vi "FPGA Acquire.vi"(0 "Logging queue in":T6, 1 "Max allowed trial length (sec)":dbl=15.0 format="%#_13g", 5 "Logging queue element IN":T3={"Imaging Protocol"=enum."Live Imaging", "Number of Trials"=0, "Frame Size"=512, "# Averaged frames"=0, "Dwell time (us)"=0.0, "Index of Z-plane"=0, "Timelapse?"=FALSE, "Logging process is active"=FALSE, "Speed logging enabled"=FALSE, "tdms file ref"=refnum, "path"=path "", "Trial Number"=0, "Expected # points acquired"=FALSE, "Manually stopped"=FALSE, "Last trial"=FALSE, "Ch0 data"=[], "Ch1 data"=[], "Ref Data"=[], "Ref Frame Time"=[], "Image Time"=[], "Continuous Time"=[], "Ref X Length"=0, "Ref Y Length"=0, "# Ref Averaged frames"=0, "Ref Dwell time (us)"=0.0, "Points acquired"={"Ch0 last trial"=0, "Ch1 last trial"=0, "All trials"=0}, "HW Timings File"=refnum} {"Ref Dwell time (us)" format="%#.6g"; "Frame Size" items=["100X100"=100, "128X128"=128, "200X200"=200, "256X256"=256, "512X512"=512, "1024x1024"=1024, "2048x2048"=2048]; "Dwell time (us)" format="%#.6g"}, 7 "FPGA Ref":T2, 9 "Target number of points":u64, 11 "error in (no error)":errorcluster, 12 "Total number of Ref points":u32, 13 "Imaging Protocol":T1) -> (4 "Logging queue out":T6, 6 "Logging queue element OUT":T3={"Imaging Protocol"=enum."Live Imaging", "Number of Trials"=0, "Frame Size"=512, "# Averaged frames"=0, "Dwell time (us)"=0.0, "Index of Z-plane"=0, "Timelapse?"=FALSE, "Logging process is active"=FALSE, "Speed logging enabled"=FALSE, "tdms file ref"=refnum, "path"=path "", "Trial Number"=0, "Expected # points acquired"=FALSE, "Manually stopped"=FALSE, "Last trial"=FALSE, "Ch0 data"=[], "Ch1 data"=[], "Ref Data"=[], "Ref Frame Time"=[], "Image Time"=[], "Continuous Time"=[], "Ref X Length"=0, "Ref Y Length"=0, "# Ref Averaged frames"=0, "Ref Dwell time (us)"=0.0, "Points acquired"={"Ch0 last trial"=0, "Ch1 last trial"=0, "All trials"=0}, "HW Timings File"=refnum} {"Ref Dwell time (us)" format="%#.6g"; "Frame Size" items=["100X100"=100, "128X128"=128, "200X200"=200, "256X256"=256, "512X512"=512, "1024x1024"=1024, "2048x2048"=2048]; "Dwell time (us)" format="%#.6g"}, 8 "Elements Remaining":u32, 10 "VI exec time":u32, 15 "error out":errorcluster)   [LabVIEW 2020]
uses:
  Typedefs/Logging queue element.ctl
  Typedefs/Imaging Protocols enum.ctl
  Typedefs/Frame Size.ctl
  Typedefs/Acquired points count.ctl
  Typedefs/Data queue ref.ctl
  RIG-SPECIFIC FILES/FPGA Refs/FPGA Ref.ctl
panel:
  out "Array":u32[](array[numeric])
  out "Ref Elements Remaining":u32
  out "# elements in queue":i32
  out "VI exec interval":u32
  out "Execution rate (Hz) 3":i32 format="Execution Rate: %.0f Hz"
  out "Execution rate (Hz)":i32 format="Execution Rate: %.0f Hz"
  out "Trial completed or \nImaging stopped":bool
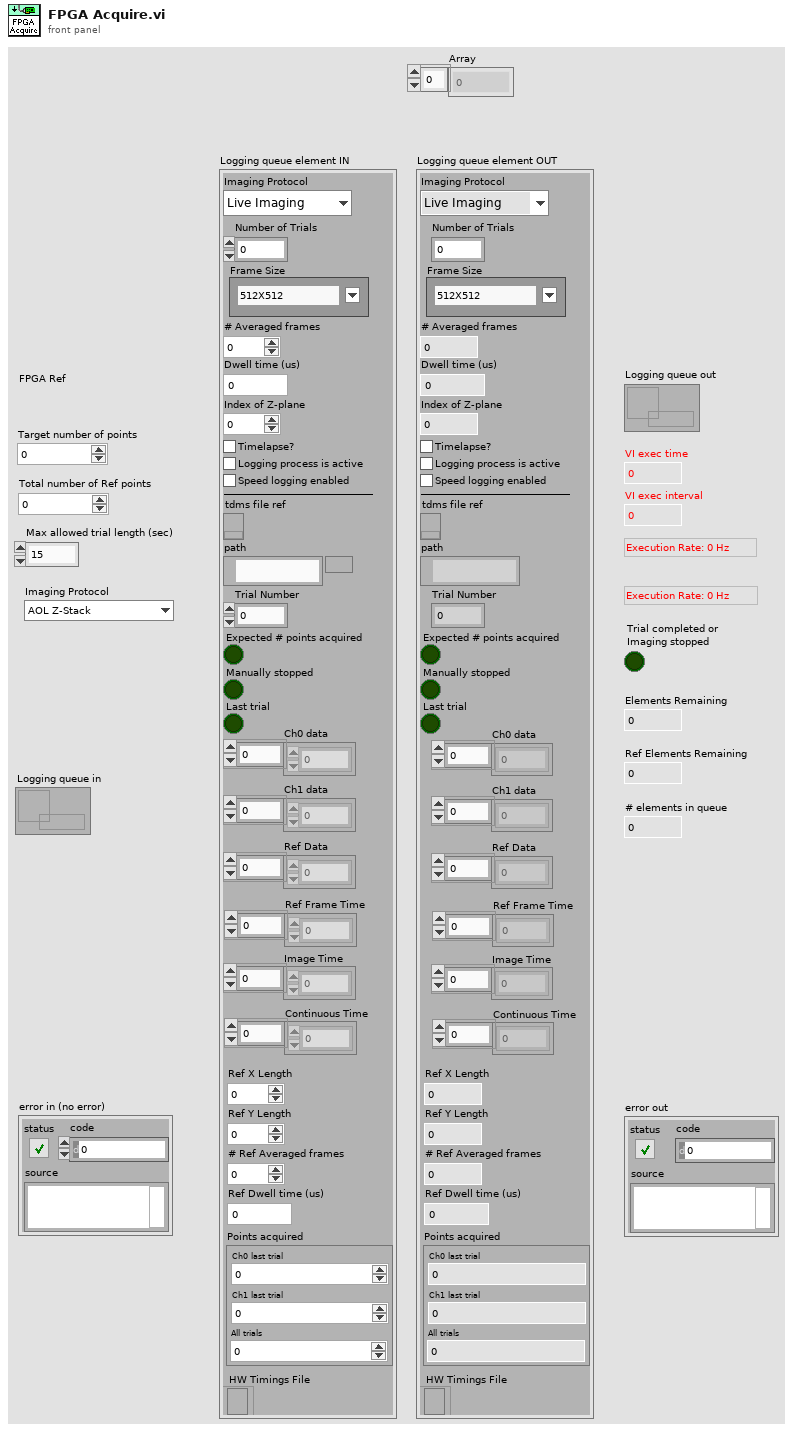
[diagram p1: front panel]
types:
  T1 = typedef "Imaging Protocols enum.ctl" = enum16{"AOL Z-Stack", "Motor Z Stack", "Functional Acquisition", "Single Plane Acquisition", "Volume Acquisition", "Live Imaging", "Live Plane Imaging", "Live Volume Imaging"}
  T2 = typedef "FPGA Ref.ctl" = refnum<k20>
  T3 = typedef "Logging queue element.ctl" = cluster{"Imaging Protocol":T1, "Number of Trials":u16, "Frame Size":T4, "# Averaged frames":u16, "Dwell time (us)":dbl, "Index of Z-plane":i32, "Timelapse?":bool, "Logging process is active":bool, "Speed logging enabled":bool, "tdms file ref":refnum<k34>, "path":path, "Trial Number":i32, "Expected # points acquired":bool, "Manually stopped":bool, "Last trial":bool, "Ch0 data":u32[], "Ch1 data":u32[], "Ref Data":u32[], "Ref Frame Time":u64[], "Image Time":u64[], "Continuous Time":u64[], "Ref X Length":u16, "Ref Y Length":u16, "# Ref Averaged frames":u16, "Ref Dwell time (us)":dbl, "Points acquired":T5, "HW Timings File":refnum<file>}
  T4 = typedef "Frame Size.ctl" = u16
  T5 = typedef "Acquired points count.ctl" = cluster{"Ch0 last trial":u64, "Ch1 last trial":u64, "All trials":u64}
  T6 = typedef "Data queue ref.ctl" = refnum<queue>
  T7 = typedef "FIFO elements available.ctl" = cluster{"Elements Available Ch0":u32, "Elements Available Ch1":u32, "Ref Elements Available":u32, "Ref Time Elements":u32, "Image Time Elements":u32, "Inter trial elements":u32, "Target number of points":u64}
  T8 = typedef "Data arrays cluster.ctl" = cluster{"Ch0 data":u32[], "Ch1 data":u32[], "Ref data":u32[], "Ref time data":u64[], "Image time data":u64[], "Continuous time data":u64[]}
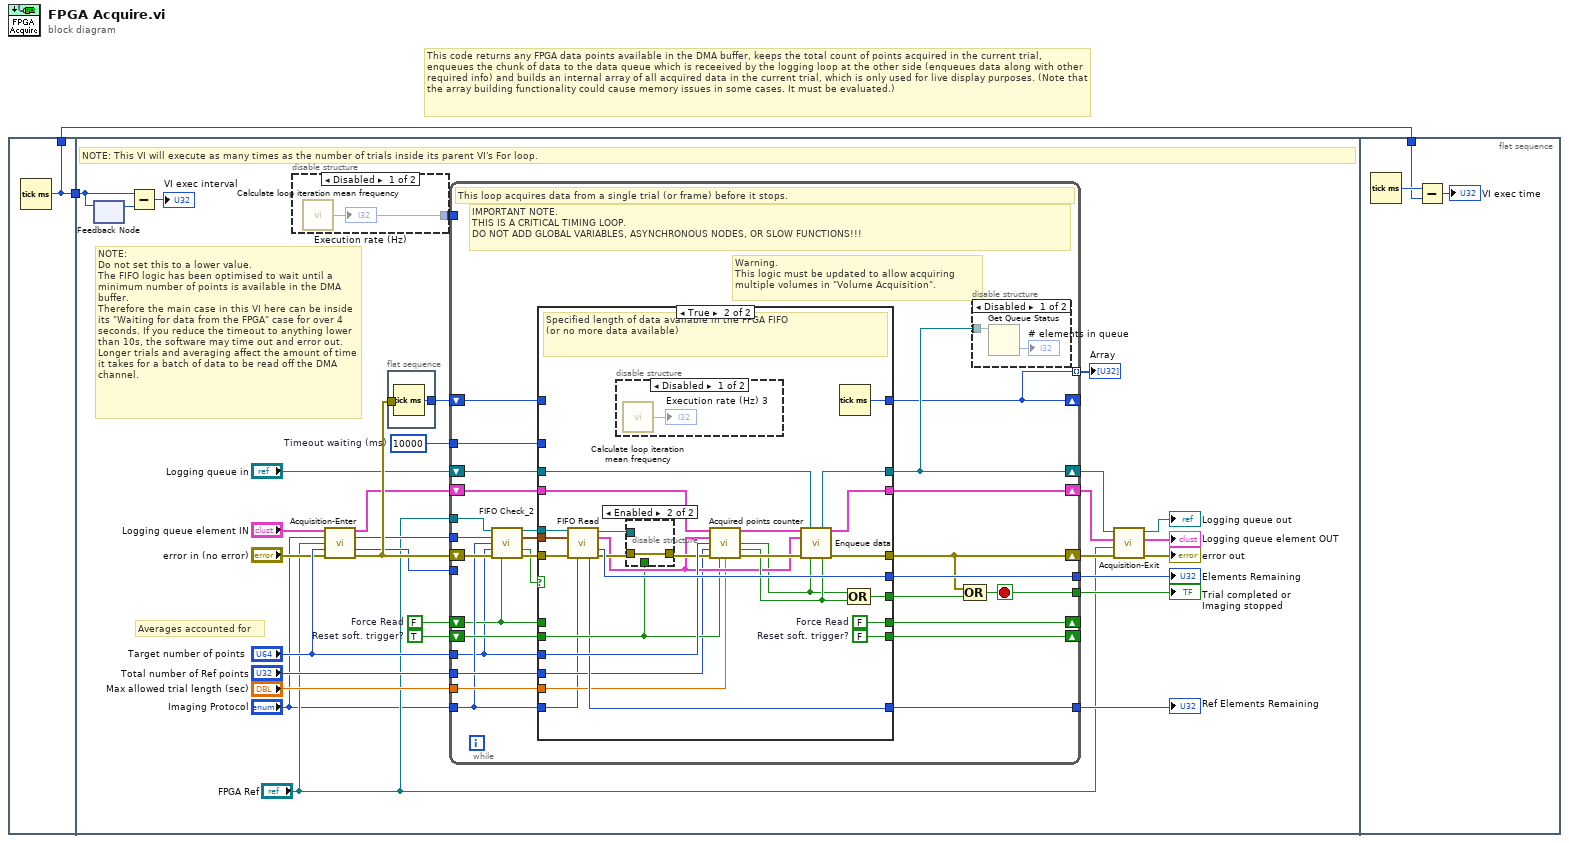
[diagram p0: block diagram]
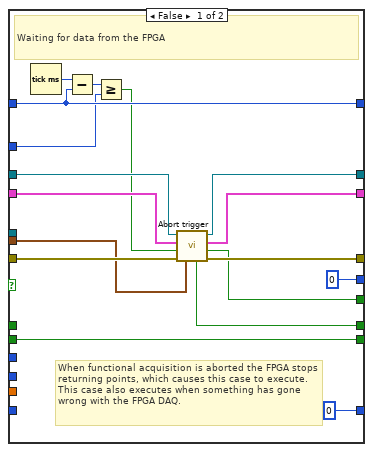
[diagram p4: hidden frame]
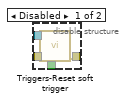
[diagram p6: hidden frame]
diagram:
  # "This code returns any FPGA data points available in the DMA buffer, keeps the total count of points acquired in the current trial, enqueues the chunk of data to the data queue which is receeived by the logging loop at the other side (enqueues data along with other required info) and builds an internal array of all acquired data in the current trial, which is only used for live display purposes. (Note that the array building functionality could cause memory issues in some cases. It must be evaluated.)"
  n1 = flat-sequence {
    tunnel: [w3] -> w1
    tunnel: [w3] -> w2
    tunnel: w2 -> [w23]
    tunnel: w1 -> [w115]
    frame #0 {
      n2 = Tick Count (ms)() -> (millisecond timer value=w3:u32)
    }
    frame #1 {
      w4 = FALSE  # Force Read
      w22 = TRUE  # Reset soft. trigger?
      w27 = u32 10000  # Timeout waiting (ms)
      # "NOTE:\nDo not set this to a lower value.\nThe FIFO logic has been optimised to wait until a minimum number of points is available in the DMA buffer.\nTherefore the main case in this VI here can be inside its \"Waiting for data from the FPGA\" case for over 4 seconds. If you reduce the timeout to anything lower than 10s, the software may time out and error out.\nLonger trials and averaging affect the amount of time it takes for a batch of data to be read off the DMA channel."
      # "Averages accounted for"
      # "NOTE: This VI will execute as many times as the number of trials inside its parent VI's For loop."
      n3 = feedback #1() -> (w25:u32)  [unwired: 1 in]
      n4 = feedback-in #1(w23) -> ()
      n5 = Subtract(x=w23, y=w25) -> (x-y=→"VI exec interval":u32)
      n6 = disable-structure "Diagram Disable Structure" shown="Disabled" {
        disable-tunnel: [w35 _] -> w26
        frame Disabled {
          n7 = call "Calculate loop iteration mean frequency.vi"() -> ("Refresh rate (Hz)"=w35:i32)  [unwired: 1 in]
          "Execution rate (Hz)" <- w35
        }
        frame Enabled {
        }
      }
      n8 = call "Acquisition-Enter.vi"("Logging queue element in"="Logging queue element IN", "Imaging Protocol"="Imaging Protocol", "FPGA Ref"="FPGA Ref", "Target number of points"="Target number of points", "error in (no error)"="error in (no error)") -> ("Logging queue element out"=w14:T3, "Read at least # points"=w21:u32, "Read at least # Ref points"=w20:u32, "error out"=w33:errorcluster)  [unwired: 7 in]
      n9 = flat-sequence {
        tunnel: [w34] -> w28
        tunnel: w33 -> [_]
        frame #0 {
          n10 = Tick Count (ms)() -> (millisecond timer value=w34:u32)
        }
      }
      n11 = while {
        tunnel: w20 -> [_]
        tunnel: [w45] -> w13
        tunnel: [w58] -> w31
        shift-right: [w51] -> w9
        shift-left: "Logging queue in" -> [w59]
        shift-right: [w43] -> w29
        shift-left: w33 -> [w62]
        tunnel: "FPGA Ref" -> [w56]
        tunnel: w26 -> [_]
        shift-right: [w39] -> _
        shift-left: w28 -> [w55]
        tunnel: w27 -> [w54]
        shift-right: [w52] -> _
        shift-left: w22 -> [w53]
        tunnel: "Target number of points" -> [w36]
        tunnel: w21 -> [w49]
        tunnel: [w48] -> w19
        tunnel: "Total number of Ref points" -> [w47]
        tunnel: "Max allowed trial length (sec)" -> [w46]
        shift-right: [w42] -> w10
        shift-left: w14 -> [w57]
        tunnel: "Imaging Protocol" -> [w40]
        tunnel: [w39] -> w5 mode=indexing
        shift-right: [w38] -> _
        shift-left: w4 -> [w37]
        stop <- w45 stop-if-true
        # "IMPORTANT NOTE.\nTHIS IS A CRITICAL TIMING LOOP.\nDO NOT ADD GLOBAL VARIABLES, ASYNCHRONOUS NODES, OR SLOW FUNCTIONS!!!"
        # "Warning.\nThis logic must be updated to allow acquiring multiple volumes in \"Volume Acquisition\"."
        # "This loop acquires data from a single trial (or frame) before it stops."
        n12 = call "FIFO Check_2.vi"("FPGA Ref in"=w56, "Read at least # points"=w49, "Imaging Protocol"=w40, "Target number of points"=w36, "error in (no error)"=w62, "Force read"=w37) -> ("FPGA Ref out"=w61:T2, "Elements Available"=w41:T7, "Data available or data has just completed (read the FIFO)"=w50:bool, "error out"=w60:errorcluster)  [unwired: 5 in, 1 out]
        n13 = case shown="True" w50 {
          tunnel: w60 -> [w75 w103]
          tunnel: w61 -> [_ w105]
          tunnel: [w67 w98] -> w44
          tunnel: w36 -> [_ w100]
          tunnel: w57 -> [w69 w90]
          tunnel: w59 -> [w73 w88]
          tunnel: [w72 w87] -> w51
          tunnel: [w76 w99] -> w43
          tunnel: [u32 0 ("Elements Remaining") w108] -> w58
          tunnel: [w71 w85] -> w42
          tunnel: w55 -> [w78 _]
          tunnel: [w78 w106] -> w39
          tunnel: w54 -> [w77 _]
          tunnel: w53 -> [w74 w94]
          tunnel: [w74 w104] -> w52
          tunnel: [u32 0 ("Ref Elements Remaining") w93] -> w48
          tunnel: w47 -> [_ w92]
          tunnel: w46 -> [_ w91]
          tunnel: w41 -> [w66 w84]
          tunnel: w40 -> [_ w83]
          tunnel: [w65 w82] -> w38
          tunnel: w37 -> [_ _]
          frame False {
            # "When functional acquisition is aborted the FPGA stops returning points, which causes this case to execute. This case also executes when something has gone wrong with the FPGA DAQ."
            # "Waiting for data from the FPGA"
            n14 = Tick Count (ms)() -> (millisecond timer value=w79:u32)
            n15 = Subtract(x=w79, y=w78) -> (x-y=w80:u32)
            n16 = Greater Or Equal?(x=w80, y=w77) -> (x >= y?=w68:bool)
            n17 = call "Abort trigger.vi"("Elements Available"=w66, "error in (no error)"=w75, "Timed out waiting on data"=w68, "Logging queue element in"=w69, "Logging queue in"=w73) -> ("error out"=w76:errorcluster, "Stop the acquisition module"=w67:bool, "Logging queue metadata shift out"=w71:T3, "Logging queue out"=w72:T6, "Force Read"=w65:bool)  [unwired: 2 in]
          }
          frame True {
            w82 = FALSE  # Force Read
            w104 = FALSE  # Reset soft. trigger?
            # "Specified length of data available in the FPGA FIFO\n(or no more data available)"
            n18 = call "FIFO Read.vi"("FPGA Ref"=w105, "Elements Available"=w84, "error in"=w103, "Imaging Protocol"=w83) -> ("FPGA VI Reference Out"=w101:T2, "Data arrays cluster"=w95:T8, "Elements Remaining (Ch0)"=w108:u32, "Image Time Elements Remaining"=w93:u32, "error out"=w102:errorcluster)  [unwired: 7 in]
            n19 = disable-structure "Diagram Disable Structure" shown="Disabled" {
              frame Disabled {
                n20 = call "Calculate loop iteration mean frequency.vi"() -> ("Refresh rate (Hz)"=→"Execution rate (Hz) 3":i32)  [unwired: 1 in]
              }
              frame Enabled {
              }
            }
            n21 = disable-structure "Diagram Disable Structure" shown="Enabled" {
              disable-tunnel: w102 -> [w113 w114]
              disable-tunnel: w101 -> [w112 _]
              disable-tunnel: [w111 w114] -> w96
              disable-tunnel: w94 -> [w110 _]
              frame Disabled {
                n22 = call "Triggers-Reset soft trigger.vi"("Reset soft. trigger"=w110, "error in (no error)"=w113, "FPGA Ref"=w112) -> ("error out"=w111:errorcluster)  [unwired: 8 in]
              }
              frame Enabled {
              }
            }
            n23 = call "Acquired points counter.vi"("Logging queue element"=w90, "Raw Data Array"=w95, "Number of samples to be acquired (points in frame x Ch. x Av.)"=w100, "Number of Ref samples to be acquired"=w92, "error in"=w96, "Initial reset"=w94, "Max allowed trial length (sec)"=w91) -> ("Logging queue element"=w86:T3, "Expected number of funct.acq points acquired on both channels"=w89:bool, "Live imaging stopped"=w97:bool, "error out"=w107:errorcluster)  [unwired: 5 in]
            n24 = call "Enqueue data.vi"("Logging queue metadata shift in"=w86, "Logging queue in"=w88, "Chunk of data"=w95, "Error in"=w107, "Expected # points acquired"=w89, "Manually stopped"=w97) -> ("Logging queue out"=w87:T6, "Logging queue metadata shift out"=w85:T3, "error out"=w99:errorcluster)  [unwired: 7 in]
            n25 = Tick Count (ms)() -> (millisecond timer value=w106:u32)
            n26 = Compound Arithmetic op=OR(w89, w97) -> (w98:bool)
          }
        }
        n27 = Compound Arithmetic op=OR(w43, w44) -> (w45:bool)
        n28 = disable-structure "Diagram Disable Structure" shown="Disabled" {
          disable-tunnel: w51 -> [w64 _]
          frame Disabled {
            n29 = Get Queue Status(queue=w64) -> (# elements in queue=→"# elements in queue":i32)  [unwired: 2 in, 7 out]
          }
          frame Enabled {
          }
        }
      }
      "Elements Remaining" <- w31
      "Trial completed or \nImaging stopped" <- w13
      "Ref Elements Remaining" <- w19
      "Array" <- w5
      n30 = call "Acquisition-Exit.vi"("error in (no error)"=w29, "FPGA Ref"="FPGA Ref", "Logging queue element in"=w10, "Logging queue in"=w9) -> ("error out"=→"error out":errorcluster, "Logging queue element"=→"Logging queue element OUT":T3, "Logging queue out"=→"Logging queue out":T6)  [unwired: 5 in]
    }
    frame #2 {
      n31 = Tick Count (ms)() -> (millisecond timer value=w116:u32)
      n32 = Subtract(x=w116, y=w115) -> (x-y=→"VI exec time":u32)
    }
  }
